vi "Evaluate Compare Group.vi"(8 "error in":errorcluster, 10 "items":T1(array[cluster]), 11 "num values":cluster{"channel":string, "value":dbl}[](array[cluster])) -> (0 "error out":errorcluster, 2 "first fail":string, 3 "passes":bool)   [LabVIEW 2026]
doc: "Compare list over numeric IO values. Every item must be found (both names) and pass its comparison: EQ/NE use the tolerance band, GT/GE/LT/LE are strict. The first failing item's name is reported."
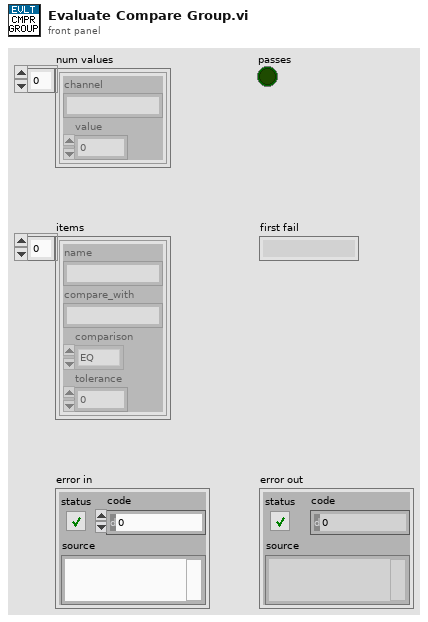
[diagram p1: front panel]
types:
  T1 = cluster{"name":string, "compare_with":string, "comparison":enum16{"EQ", "NE", "GT", "GE", "LT", "LE"}, "tolerance":dbl}[]
  T2 = cluster{"name":string, "compare_with":string, "comparison":enum16{"EQ", "NE", "GT", "GE", "LT", "LE"}, "tolerance":dbl}
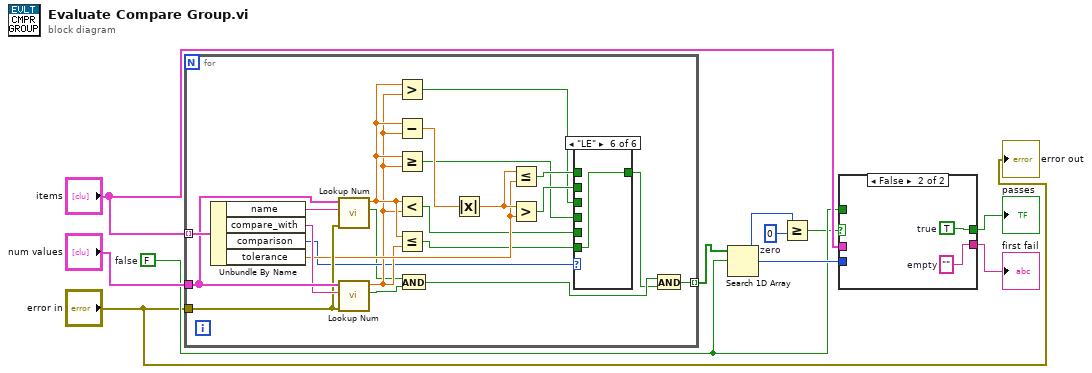
[diagram p0: block diagram]
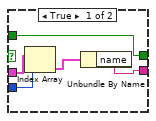
[diagram p2: hidden frame]
diagram:
  w8 = 0  # zero
  w5 = FALSE  # false
  n1 = for {
    tunnel: "items" -> [w32] mode=indexing
    tunnel: "num values" -> [w30]
    tunnel: "error in" -> [w28]
    tunnel: [w11] -> w9 mode=indexing
    n2 = Unbundle By Name(w32) -> ("name"=w31:string, "compare_with"=w29:string, "comparison"=w16:enum16{"EQ", "NE", "GT", "GE", "LT", "LE"}, "tolerance"=w25:dbl)
    n3 = call "Lookup Num.vi"("error in"=w28, "name"=w31, "num values"=w30) -> ("found"=w15:bool, "value"=w24:dbl)  [unwired: 6 in, 1 out]
    n4 = call "Lookup Num.vi"("error in"=w28, "name"=w29, "num values"=w30) -> ("found"=w14:bool, "value"=w23:dbl)  [unwired: 6 in, 1 out]
    n5 = Greater?(x=w24, y=w23) -> (0:w20:bool)
    n6 = Subtract(x=w24, y=w23) -> (x-y=w27:dbl)
    n7 = Greater Or Equal?(x=w24, y=w23) -> (x >= y?=w19:bool)
    n8 = Less?(x=w24, y=w23) -> (x < y?=w18:bool)
    n9 = Less Or Equal?(x=w24, y=w23) -> (x <= y?=w17:bool)
    n10 = And(x=w15, y=w14) -> (x .and. y?=w13:bool)
    n11 = Absolute Value(x=w27) -> (abs(x)=w26:dbl)
    n12 = Less Or Equal?(x=w26, y=w25) -> (x <= y?=w22:bool)
    n13 = Greater?(x=w26, y=w25) -> (0:w21:bool)
    n14 = case shown="\"LE\"" w16 {
      tunnel: w22 -> [w33 _ _ _ _ _]
      tunnel: w21 -> [_ w34 _ _ _ _]
      tunnel: w20 -> [_ _ w35 _ _ _]
      tunnel: w19 -> [_ _ _ w36 _ _]
      tunnel: w18 -> [_ _ _ _ w37 _]
      tunnel: w17 -> [_ _ _ _ _ w38]
      tunnel: [w33 w34 w35 w36 w37 w38] -> w12
      frame "EQ" {
      }
      frame "NE" {
      }
      frame "GT" {
      }
      frame "GE" {
      }
      frame "LT" {
      }
      frame "LE" {
      }
    }
    n15 = And(x=w13, y=w12) -> (x .and. y?=w11:bool)
  }
  n16 = Search 1D Array(1D array=w9, element=w5) -> (index of element=w6:i32)  [unwired: 1 in]
  n17 = Greater Or Equal?(x=w6, y=w8) -> (x >= y?=w4:bool)
  n18 = case shown="False" w4 {
    tunnel: "items" -> [w43 _]
    tunnel: w6 -> [w42 _]
    tunnel: [w40 w45] -> w3
    tunnel: w5 -> [w40 _]
    tunnel: [w39 w44] -> w2
    frame True {
      n19 = Index Array(array=w43, index=w42) -> (element=w41:T2)
      n20 = Unbundle By Name(w41) -> ("name"=w39:string)
    }
    frame False {
      w44 = ""  # empty
      w45 = TRUE  # true
    }
  }
  "passes" <- w3
  "first fail" <- w2
  "error out" <- "error in"
